vi "Connect.vi"(8 "error in (no error)":errorcluster, 10 "Connection String":string, 11 "MySqlConnection in":refnum<class "DBC.lvclass">) -> (0 "error out":errorcluster, 3 "MySqlConnection out":refnum<class "DBC.lvclass">)   [LabVIEW 2026, in "ORM_DBC_MySql_netCore.lvlib" / "DBC.lvclass"]
uses:
  DBC.lvclass
  C:/Viviota/Projects/R&D/__OpenSource/labview-orm/libraries_netcore/MySqlConnector.dll
  libraries_netcore/MySqlConnector.dll
  <vilib>/Viviota/shared/ORM_DBC_dotNetCore.lvlibp/Write connection.vi
  <vilib>/Viviota/shared/ORM.lvlibp/DbConnection/Write ColumnNameEqualsValueFormat.vi
  <vilib>/Viviota/shared/ORM.lvlibp/DbConnection/Write ColumnNameFormat.vi
  <vilib>/Viviota/shared/ORM.lvlibp/DbConnection/Write LastIdentityQuery.vi
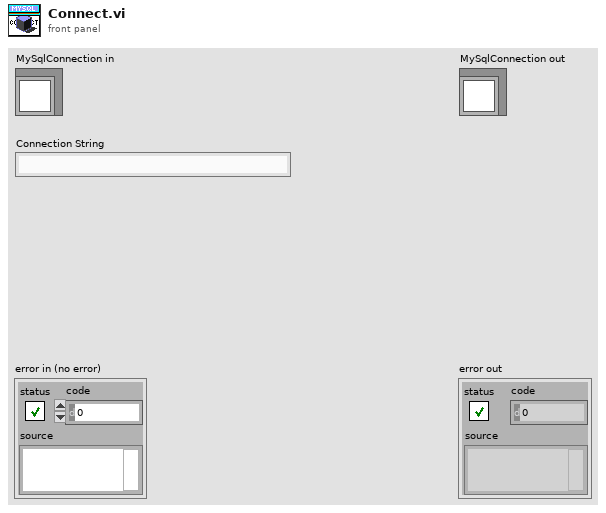
[diagram p1: front panel]
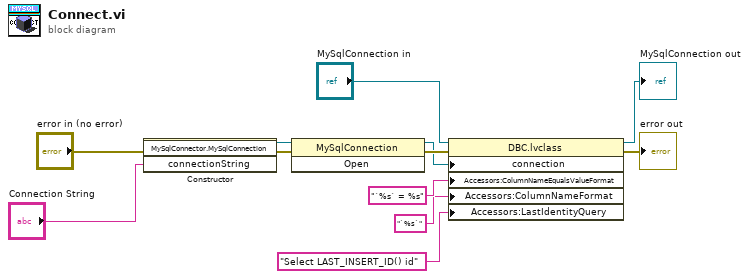
[diagram p0: block diagram]
diagram:
  n1 = constructor class="MySqlConnection"(error in="error in (no error)", "connectionString"="Connection String") -> (reference out=w9:refnum<k39>, error out=w10:errorcluster)  [unwired: 2 in, 2 out]
  n2 = invoke class="MySqlConnection" method="Open"(reference=w9, error in=w10) -> (reference out=w11:refnum<k39>, error out=w12:errorcluster)  [unwired: 1 in, 1 out]
  n3 = property class="DBC.lvclass"(reference="MySqlConnection in", error in=w12, "connection"=w11, "Accessors:ColumnNameEqualsValueFormat"="`%s` = %s" ("ColumnNameFormat"), "Accessors:ColumnNameFormat"="`%s`" ("ColumnNameFormat"), "Accessors:LastIdentityQuery"="Select LAST_INSERT_ID() id" ("LastIdentityQuery")) -> (reference out=→"MySqlConnection out":refnum<class "DBC.lvclass">, error out=→"error out":errorcluster)
